vi "VIs Filter Controls.vi"(9 "ControlsFilter":T2={"VI.Filter.Label"="num", "VI.Filter.Class"="", "No Error Cluster"=TRUE, "NonTranslated"=TRUE, "OnlyVisibleArea"=TRUE} caption="Controls Filter:", 10 "VIs":map{path, T1[]}(c390), 11 "Path":path) -> (3 "Filtered Ctrls":T1[](array[typedef]))   [LabVIEW 2019, in "Language Editor.lvlib"]
doc: "- - -\nCopyright (c) 2026, Merecs Engineering GmbH"
uses:
  Language Editor.lvlib
  type defs/Cluster VI controls.ctl
panel:
  # "Connector Pane"
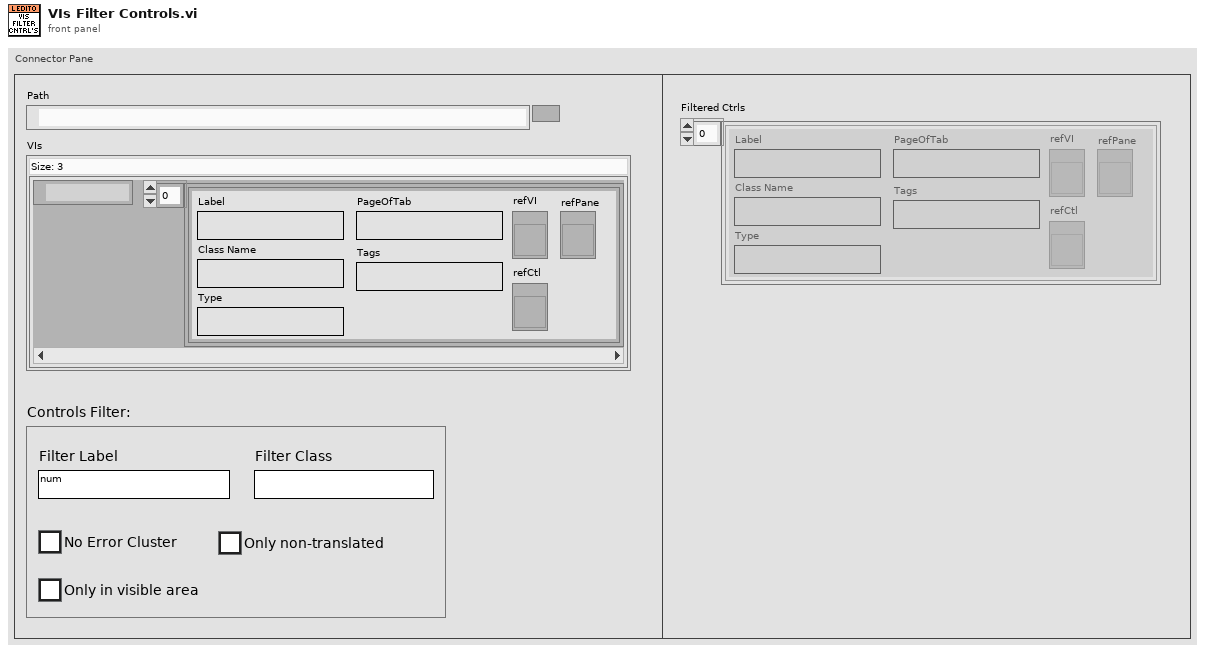
[diagram p1: front panel]
types:
  T1 = typedef "Language Editor.lvlib/Cluster VI controls.ctl" = cluster{"Label":string, "Class Name":string, "Type":string, "Tags":string, "refVI":refnum<vi>, "refCtl":refnum<vi>, "PageOfTab":string, "refPane":refnum<vi>}
  T2 = cluster{"VI.Filter.Label":string, "VI.Filter.Class":string, "No Error Cluster":bool, "NonTranslated":bool, "OnlyVisibleArea":bool}
  T3 = typedef "LVRectTypeDef.ctl" = cluster{"Left":i16, "Top":i16, "Right":i16, "Bottom":i16}
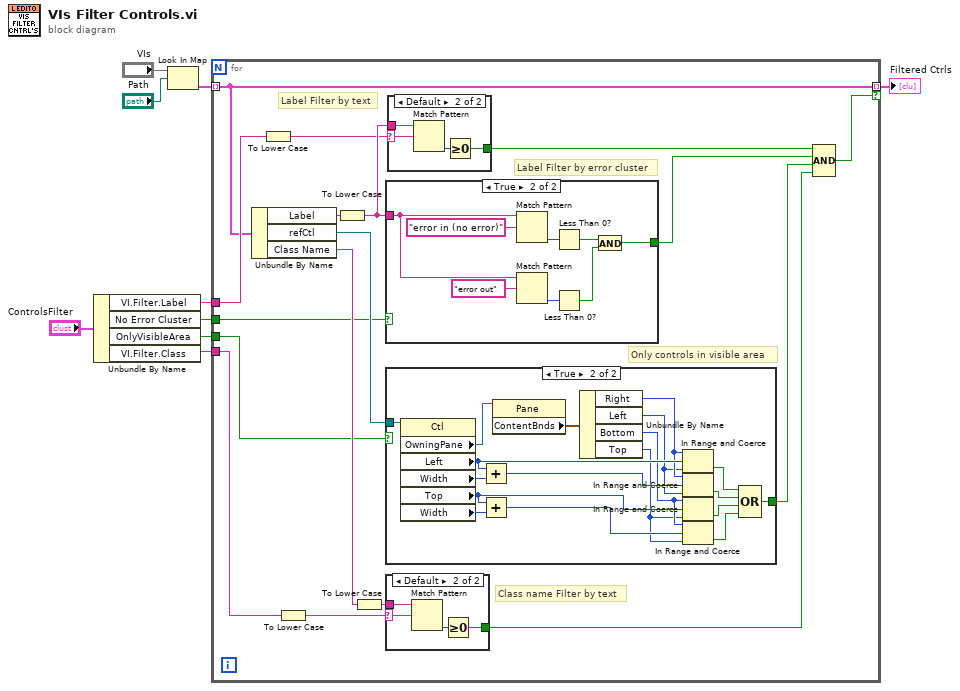
[diagram p0: block diagram]
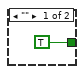
[diagram p2: hidden frame]
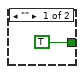
[diagram p3: hidden frame]
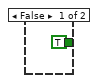
[diagram p4: hidden frame]
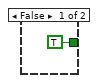
[diagram p5: hidden frame]
diagram:
  n1 = Unbundle By Name("ControlsFilter") -> ("VI.Filter.Label"=w1:string, "No Error Cluster"=w5:bool, "OnlyVisibleArea"=w4:bool, "VI.Filter.Class"=w2:string)
  n2 = Look In Map(map="VIs", key="Path") -> (value=w6:T1[])  [unwired: 1 in, 1 out]
  n3 = for {
    tunnel: w6 -> [w22] mode=indexing
    tunnel: w5 -> [w21]
    tunnel: w4 -> [w20]
    tunnel: [w22] -> w3 mode=indexing if=w15
    tunnel: w1 -> [w23]
    tunnel: w2 -> [w19]
    # "Class name Filter by text"
    # "Only controls in visible area"
    # "Label Filter by error cluster"
    # "Label Filter by text"
    n4 = Unbundle By Name(w22) -> ("Label"=w24:string, "refCtl"=w26:refnum<vi>, "Class Name"=w25:string)
    n5 = To Lower Case(string=w23) -> (all lower case string=w10:string)
    n6 = To Lower Case(string=w19) -> (all lower case string=w13:string)
    n7 = To Lower Case(string=w24) -> (all lower case string=w11:string)
    n8 = To Lower Case(string=w25) -> (all lower case string=w12:string)
    n9 = case shown="True" w21 {
      tunnel: w11 -> [_ w62]
      tunnel: [TRUE w57] -> w18
      frame False {
      }
      frame True {
        n10 = Match Pattern(string=w62, regular expression="error in (no error)") -> (offset past match=w64:i32)  [unwired: 1 in, 3 out]
        n11 = Match Pattern(string=w62, regular expression="error out") -> (offset past match=w60:i32)  [unwired: 1 in, 3 out]
        n12 = Less Than 0?(x=w64) -> (x < 0?=w59:bool)
        n13 = Less Than 0?(x=w60) -> (x < 0?=w58:bool)
        n14 = And(x=w59, y=w58) -> (x .and. y?=w57:bool)
      }
    }
    n15 = case shown="True" w20 {
      tunnel: [TRUE w38] -> w17
      tunnel: w26 -> [_ w55]
      frame False {
      }
      frame True {
        n16 = property class="Ctl"(reference=w55) -> ("OwningPane"=w48:refnum<vi>, "Left"=w52:i32, "Width"=w54:u32, "Top"=w51:i32, "Width"=w53:u32)  [unwired: 1 in, 2 out]
        n17 = Add(x=w52, y=w54) -> (x+y=w50:u32)
        n18 = Add(x=w51, y=w53) -> (x+y=w49:u32)
        n19 = property class="Pane"(reference=w48) -> ("ContentBnds"=w47:T3)  [unwired: 1 in, 2 out]
        n20 = Unbundle By Name(w47) -> ("Right"=w46:i16, "Left"=w45:i16, "Bottom"=w44:i16, "Top"=w43:i16)
        n21 = In Range and Coerce(upper limit=w46, x=w52, lower limit=w45) -> (In Range?=w42:bool)  [unwired: 1 out]
        n22 = In Range and Coerce(upper limit=w46, x=w50, lower limit=w45) -> (In Range?=w41:bool)  [unwired: 1 out]
        n23 = In Range and Coerce(upper limit=w44, x=w51, lower limit=w43) -> (In Range?=w40:bool)  [unwired: 1 out]
        n24 = In Range and Coerce(upper limit=w44, x=w49, lower limit=w43) -> (In Range?=w39:bool)  [unwired: 1 out]
        n25 = Compound Arithmetic op=OR(w42, w41, w40, w39) -> (w38:bool)
      }
    }
    n26 = case shown="Default" w13 {
      selector: w13 -> [_ w30]
      tunnel: w12 -> [_ w31]
      tunnel: [TRUE w28] -> w16
      frame "" {
      }
      frame Default {
        n27 = Match Pattern(string=w31, regular expression=w30) -> (offset past match=w29:i32)  [unwired: 1 in, 3 out]
        n28 = Greater Or Equal To 0?(x=w29) -> (x >= 0?=w28:bool)
      }
    }
    n29 = case shown="Default" w10 {
      selector: w10 -> [_ w35]
      tunnel: w11 -> [_ w36]
      tunnel: [TRUE w33] -> w14
      frame "" {
      }
      frame Default {
        n30 = Match Pattern(string=w36, regular expression=w35) -> (offset past match=w34:i32)  [unwired: 1 in, 3 out]
        n31 = Greater Or Equal To 0?(x=w34) -> (x >= 0?=w33:bool)
      }
    }
    n32 = Compound Arithmetic op=AND(w14, w18, w17, w16) -> (w15:bool)
  }
  "Filtered Ctrls" <- w3
